vi "Read.vi"(8 "error in (no error)":errorcluster, 11 "HANDLE":u32) -> (0 "error out":errorcluster, 1 "BUFFER":u8[](array[numeric]), 3 "OUT":i32)   [LabVIEW 2011, in "HID_ARZ.lvlib"]
doc: "READ Read;"
uses:
  HID_ARZ.lvlib
  <userlib>/HID_ARZ/mcHID.dll
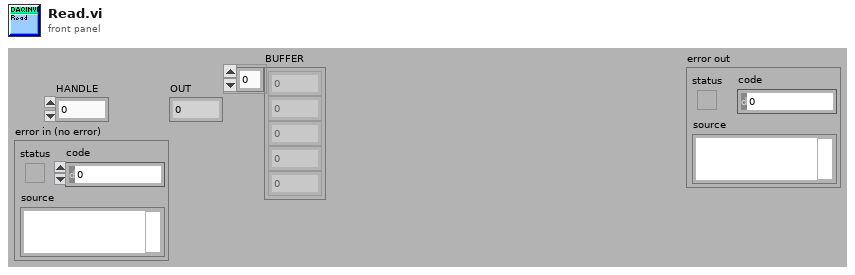
[diagram p1: front panel]
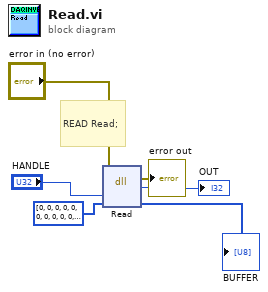
[diagram p0: block diagram]
diagram:
  # "READ Read;"
  n1 = dll-call lib="C:/Program Files (x86)/National Instruments/LabVIEW 2017/user.lib/HID_ARZ/mcHID.dll" fn="Read"(error in="error in (no error)", "HANDLE"="HANDLE", "BUFFER"=u8[] [0, 0, 0, 0, 0, 0, 0, 0, 0, 0, 0, 0, 0, 0, 0, 0, 0, 0, 0, 0, 0, 0, 0, 0, 0, 0, 0, 0, 0, 0, 0, 0, 0, 0, 0, 0, 0, 0, 0, 0, 0, 0, 0, 0, 0, 0, 0, 0, 0, 0, 0, 0, 0, 0, 0, 0, 0, 0, 0, 0, 0, 0, 0, 0]) -> (error out=→"error out":errorcluster, "return type"=→"OUT":i32, "BUFFER"=→"BUFFER":u8[])  [unwired: 3 in, 1 out]
